vi "log_recording.vi"(8 "error in":errorcluster, 9 "日志内容":string, 10 "日志选择":T1) -> (0 "error out":errorcluster)   [LabVIEW 2018, in "Log_class.lvlib"]
doc: "这是一个外部交互（写入）的日志接口\n\n_____\nCreated using DQMH Framework: Event Scripter 7.1.1.1528."
uses:
  Log_class.lvlib
  Register_logs.ctl
  Log recording Argument--cluster.ctl
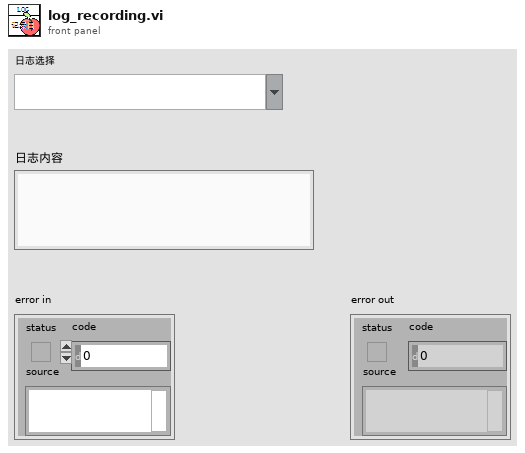
[diagram p1: front panel]
types:
  T1 = typedef "Log_class.lvlib/Register_logs.ctl" = string
  T2 = typedef "Log_class.lvlib/Log recording Argument--cluster.ctl" = cluster{"日志选择":T1, "日志内容":string}
  T3 = typedef "Log_class.lvlib/Request Events--cluster.ctl" = cluster{"Stop Module":refnum<user-event>, "Show Panel":refnum<user-event>, "Hide Panel":refnum<user-event>, "Get Module Execution Status":refnum<user-event>, "Show Diagram":refnum<user-event>, "记录日志":refnum<user-event>, "存储方式更改":refnum<user-event>, "请求日志":refnum<user-event>, "请求保存":refnum<user-event>}
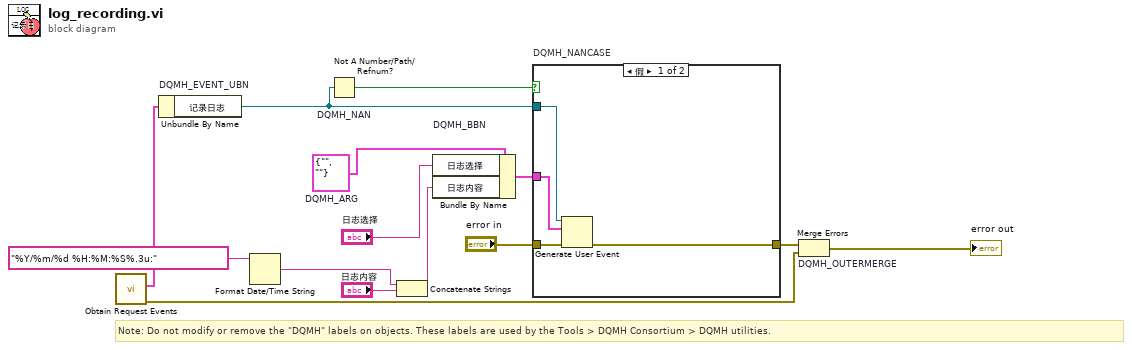
[diagram p0: block diagram]
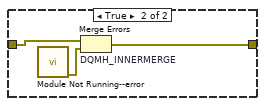
[diagram p2: hidden frame]
diagram:
  w8 = T2 {"日志选择"="", "日志内容"=""}  # DQMH_ARG
  # "Note: Do not modify or remove the \"DQMH\" labels on objects. These labels are used by the Tools > DQMH Consortium > DQMH utilities."
  n1 = call "Obtain Request Events.vi"() -> ("error out"=w6:errorcluster, "模块化日志 Request Events"=w5:T3)  [unwired: 10 in]
  n2 = Unbundle By Name "DQMH_EVENT_UBN"(w5) -> ("记录日志"=w10:refnum<user-event>)
  n3 = Format Date/Time String(time format string (%c)="%Y/%m/%d %H:%M:%S%.3u:" ("时间格式字符串(%c)")) -> (date/time string=w2:string)  [unwired: 2 in]
  n4 = Not A Number/Path/Refnum? "DQMH_NAN"(number/path/refnum=w10) -> (NaN/Path/Refnum?=w11:bool)
  n5 = Concatenate Strings(w2, "日志内容") -> (w1:string)
  n6 = Bundle By Name "DQMH_BBN"(cluster=w8, "日志选择"="日志选择", "日志内容"=w1) -> (w12:T2)
  n7 = case "DQMH_NANCASE" shown="假" w11 {
    tunnel: "error in" -> [w18 w21]
    tunnel: [w17 w20] -> w9
    tunnel: w10 -> [w16 _]
    tunnel: w12 -> [w15 _]
    frame False {
      n8 = Generate User Event(user event=w16, event data cluster=w15, error in=w18) -> (error out=w17:errorcluster)  [unwired: 1 in, 1 out]
    }
    frame True {
      n9 = call "Module Not Running--error.vi"() -> ("error out"=w19:errorcluster)  [unwired: 11 in]
      n10 = Merge Errors "DQMH_INNERMERGE"(w21, w19) -> (w20:errorcluster)
    }
  }
  n11 = Merge Errors "DQMH_OUTERMERGE"(w9, w6) -> (→"error out":errorcluster)
